vi "WriteDirection.vi"(8 "error in (no error)":errorcluster, 10 "Direction":T1, 11 "object in":refnum<class "DIO-Configuration.lvclass">) -> (0 "error out":errorcluster, 3 "object out":refnum<class "DIO-Configuration.lvclass">)   [LabVIEW 2021, in "DIO-Channel.lvlib" / "DIO-Configuration.lvclass"]
uses:
  DIO-Configuration.lvclass
  tdef/Direction.ctl
  DIO-Configuration.lvclass/DIO-Configuration.ctl
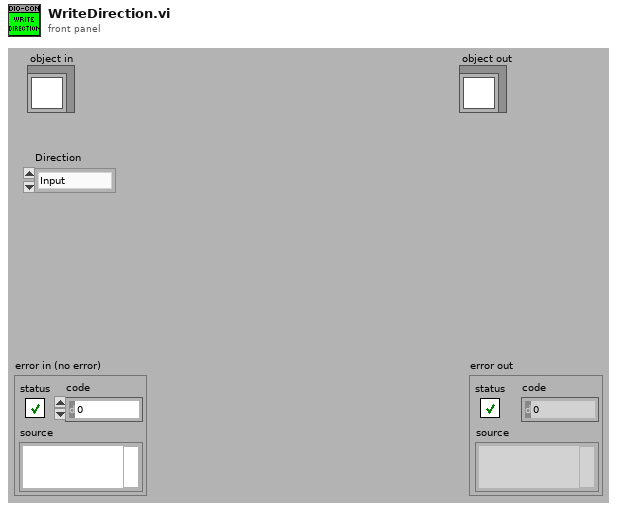
[diagram p1: front panel]
types:
  T1 = typedef "DIO-Channel.lvlib/DIO-Configuration.lvclass/Direction.ctl" = enum16{"Input", "Output"}
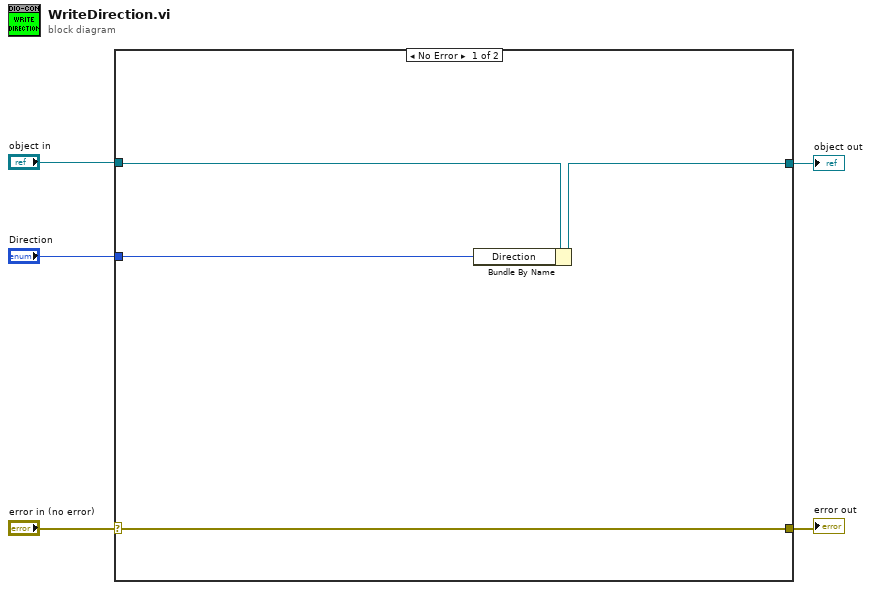
[diagram p0: block diagram]
diagram:
  n1 = case shown="No Error" "error in (no error)" {
    selector: "error in (no error)" -> [w8 w11]
    tunnel: [w8 w11] -> w4
    tunnel: [w6 w10] -> w2
    tunnel: "object in" -> [w7 w10]
    tunnel: "Direction" -> [w9 _]
    frame No Error {
      n2 = Bundle By Name(cluster=w7, "Direction"=w9) -> (w6:refnum<class "DIO-Configuration.lvclass">)
    }
    frame Error {
    }
  }
  "error out" <- w4
  "object out" <- w2
